vi "Ecrire Alarmes MODBUS EPC.vi"(1 "Adresse rég":u8 caption="Adresse régulateur", 2 "Programmation configuration":cluster{"Command (PV)":string, dbl}[](array[cluster]), 3 "Port COM run 1 REG":refnum<visa-resource-name>) -> (0 "error out":errorcluster caption="error IO")   [LabVIEW 2022 SP3]
uses:
  Variables globales/Variables glob EUROTHERM.vi
panel:
  out "Alarme haute":dbl
  out "Alarme basse":dbl
  out "Nom rég":string caption="Nom régulateur"
  in  "error in":errorcluster caption="error IO"
  # "écrire alarmes"
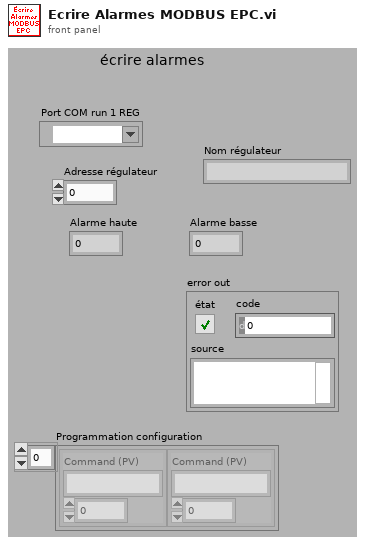
[diagram p1: front panel]
types:
  T1 = typedef "Semaphore RefNum" = refnum<k1>
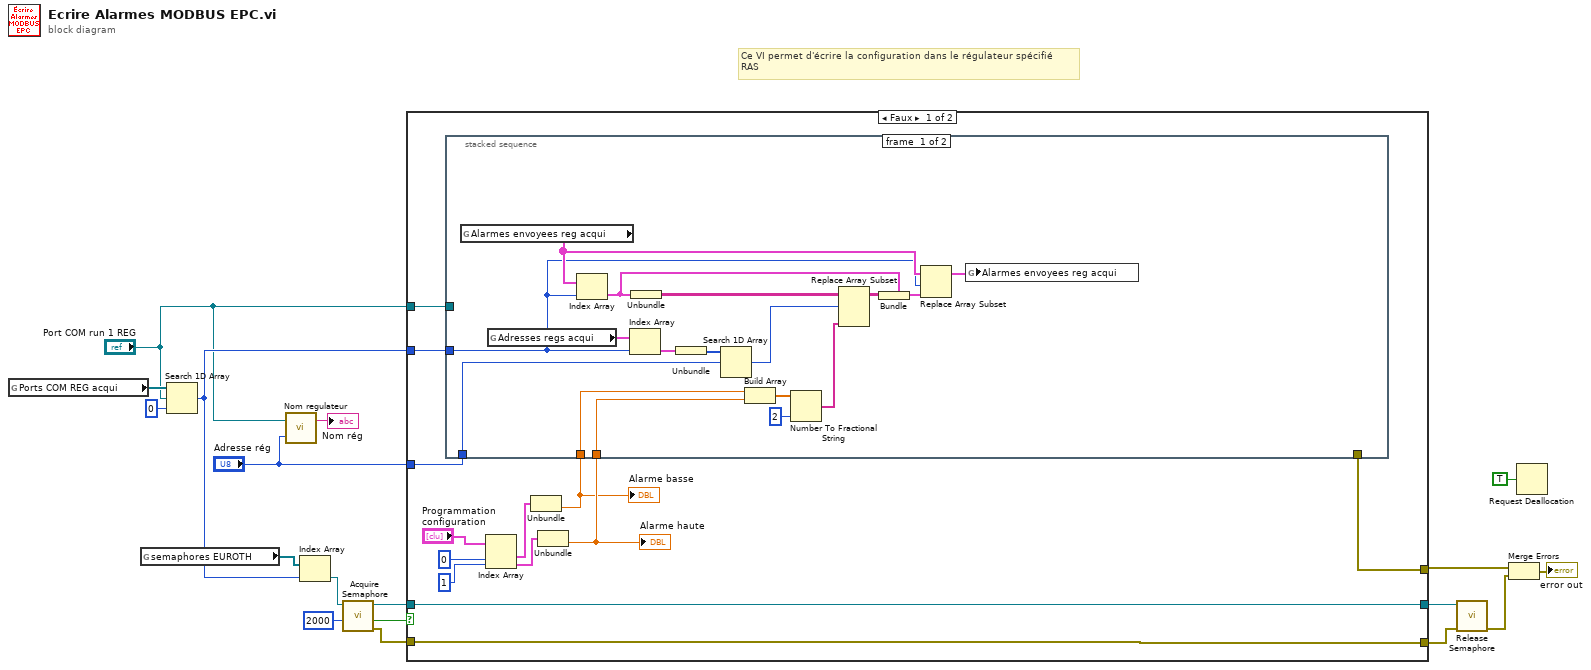
[diagram p0: block diagram]
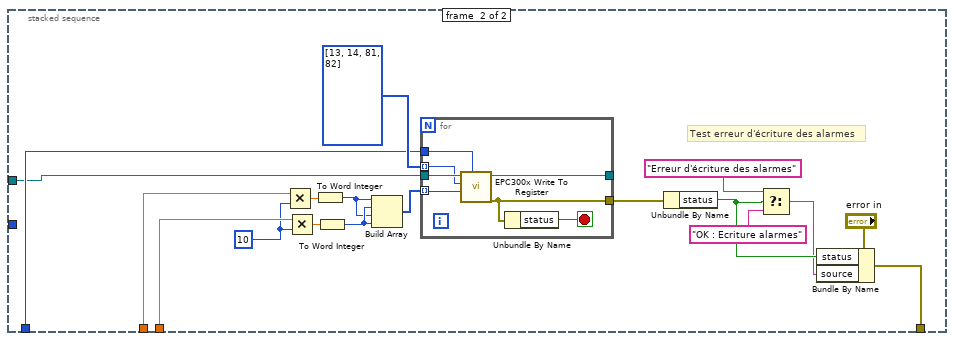
[diagram p2: hidden frame]
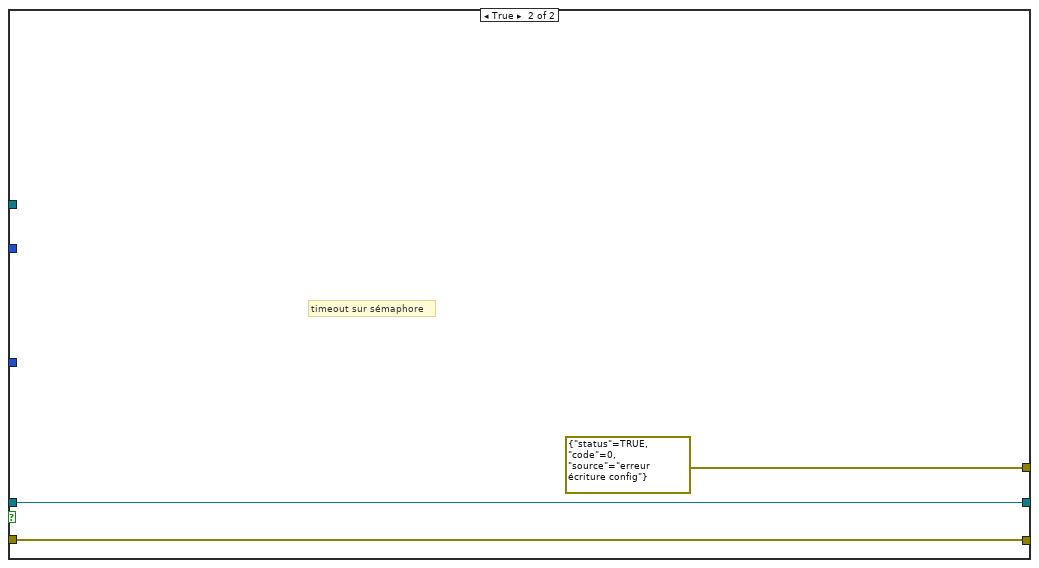
[diagram p3: hidden frame]
diagram:
  # "Ce VI permet d'écrire la configuration dans le régulateur spécifié\nRAS"
  n1 = global read "Variables glob EUROTHERM.vi" "Ports COM REG acqui"() -> (w4:refnum<visa-resource-name>[])
  n2 = global read "Variables glob EUROTHERM.vi" "semaphores EUROTH"() -> (w8:T1[])
  n3 = Search 1D Array(1D array=w4, element="Port COM run 1 REG", start index (0)=0 ("indice de départ (0)")) -> (index of element=w2:i32)
  n4 = call "Nom regulateur.vi"("Adresse régulateur"="Adresse rég", "Port COM run 1 REG"="Port COM run 1 REG") -> ("Nom régulateur"=→"Nom rég":string)  [unwired: 1 in]
  n5 = Index Array(array=w8, index=w2) -> (element=w7:T1)
  n6 = call <vilib>:"Acquire Semaphore.vi"("ms timeout (-1)"=2000, "semaphore"=w7) -> ("error out"=w13:errorcluster, "timed out"=w17:bool, "semaphore out"=w15:T1)  [unwired: 3 in]
  n7 = case shown="Faux" w17 {
    tunnel: [w26 w76] -> w14
    tunnel: w15 -> [w26 w76]
    tunnel: w13 -> [w25 w75]
    tunnel: [w25 w75] -> w12
    tunnel: [w22 errorcluster {"status"=TRUE, "code"=0, "source"="erreur écriture config"} ("error in")] -> w10
    tunnel: "Port COM run 1 REG" -> [w21 _]
    tunnel: "Adresse rég" -> [w24 _]
    tunnel: w2 -> [w23 _]
    frame False {
      n8 = Index Array(array="Programmation configuration", index #1=0 ("indice"), index #2=1 ("indice")) -> (element #1=w30:cluster{"Command (PV)":string, dbl}, element #2=w31:cluster{"Command (PV)":string, dbl})
      n9 = Unbundle(w30) -> (w19:dbl)  [unwired: 1 out]
      "Alarme basse" <- w19
      n10 = Unbundle(w31) -> (w20:dbl)  [unwired: 1 out]
      "Alarme haute" <- w20
      n11 = stacked-sequence {
        tunnel: w24 -> [w45 w58]
        tunnel: w19 -> [w42 w52]
        tunnel: w23 -> [w34 _]
        tunnel: [_ w61] -> w22
        tunnel: w21 -> [_ w57]
        tunnel: w20 -> [w32 w55]
        frame #0 {
          n12 = global read "Variables glob EUROTHERM.vi" "Alarmes envoyees reg acqui"() -> (w36:cluster{"alarmes 1COM reg":string[][]}[])
          n13 = global read "Variables glob EUROTHERM.vi" "Adresses regs acqui"() -> (w48:cluster{"Adresses acqui 1COM reg":u16[]}[])
          n14 = Index Array(array=w36, index=w34) -> (element=w37:cluster{"alarmes 1COM reg":string[][]})
          n15 = Index Array(array=w48, index=w34) -> (element=w47:cluster{"Adresses acqui 1COM reg":u16[]})
          n16 = Unbundle(w37) -> ("alarmes 1COM reg"=w44:string[][])
          n17 = Unbundle(w47) -> ("Adresses acqui 1COM reg"=w46:u16[])
          n18 = Search 1D Array(1D array=w46, element=w45) -> (index of element=w43:i32)  [unwired: 1 in]
          n19 = Build Array(w42, w32) -> (w41:dbl[])
          n20 = Number To Fractional String(number=w41, precision (6)=i16 2 ("précision (6)")) -> (F-format string=w40:string[])  [unwired: 2 in]
          n21 = Replace Array Subset(array=w44, new element=w40, index (row)=w43) -> (w38:string[][])  [unwired: 1 in]
          n22 = Bundle(cluster=w37, "alarmes 1COM reg"=w38) -> (w35:cluster{"alarmes 1COM reg":string[][]})
          n23 = Replace Array Subset(array=w36, new element=w35, index=w34) -> (w33:cluster{"alarmes 1COM reg":string[][]}[])
          n24 = global write "Variables glob EUROTHERM.vi" "Alarmes envoyees reg acqui"(w33) -> ()
        }
        frame #1 {
          w49 = i16 10 ("y")
          # "Test erreur d'écriture des alarmes"
          n25 = Multiply(x=w52, y=w49) -> (x*y=w51:dbl)
          n26 = Multiply(x=w55, y=w49) -> (x*y=w54:dbl)
          n27 = To Word Integer(number=w51) -> (16bit integer=w50:i16)
          n28 = To Word Integer(number=w54) -> (16bit integer=w53:i16)
          n29 = Build Array(w50, w53, w50, w53) -> (w60:i16[])
          n30 = for {
            tunnel: [w73] -> _
            tunnel: [w72] -> w56
            tunnel: w58 -> [w71]
            tunnel: w57 -> [w70]
            tunnel: u16[] [13, 14, 81, 82] ("Registers Addresses (0) 2") -> [w69] mode=indexing
            tunnel: w60 -> [w68] mode=indexing
            stop <- w67 stop-if-true
            n31 = call "EPC300x Write To Register.vi"("Unit Address (1)"=w71, "Data (0)"=w68, "Register Address (0)"=w69, "VISA session"=w70) -> ("error out"=w72:errorcluster, "dup VISA session"=w73:refnum<visa-resource-name>)  [unwired: 6 in]
            n32 = Unbundle By Name(w72) -> ("status"=w67:bool)
          }
          n33 = Unbundle By Name(w56) -> ("status"=w66:bool)
          n34 = Select(t="Erreur d'écriture des alarmes", s=w66, f="OK : Ecriture alarmes") -> (s? t:f=w65:string)
          n35 = Bundle By Name(cluster="error in", "status"=w66, "source"=w65) -> (w61:errorcluster)
        }
      }
    }
    frame True {
      # "timeout sur sémaphore"
    }
  }
  n36 = call <vilib>:"Release Semaphore.vi"("error in (no error)"=w12, "semaphore"=w14) -> ("error out"=w9:errorcluster)  [unwired: 4 in, 1 out]
  n37 = Merge Errors(w10, w9) -> (→"error out":errorcluster)
  n38 = Request Deallocation(TRUE ("flag")) -> ()
